vi "Read Instrument.vi"(8 "error in (no error)":errorcluster, 11 "Submodule EOL configuration in":refnum<class "Submodule EOL configuration.lvclass">) -> (0 "error out":errorcluster, 2 "Instrument":T1, 3 "Submodule EOL configuration out":refnum<class "Submodule EOL configuration.lvclass">)   [LabVIEW 2025, in "Submodule EOL.lvlib" / "Submodule EOL configuration.lvclass"]
uses:
  Submodule EOL configuration.lvclass
  Instrumnet.ctl
  Submodule EOL configuration.lvclass/Submodule EOL configuration.ctl
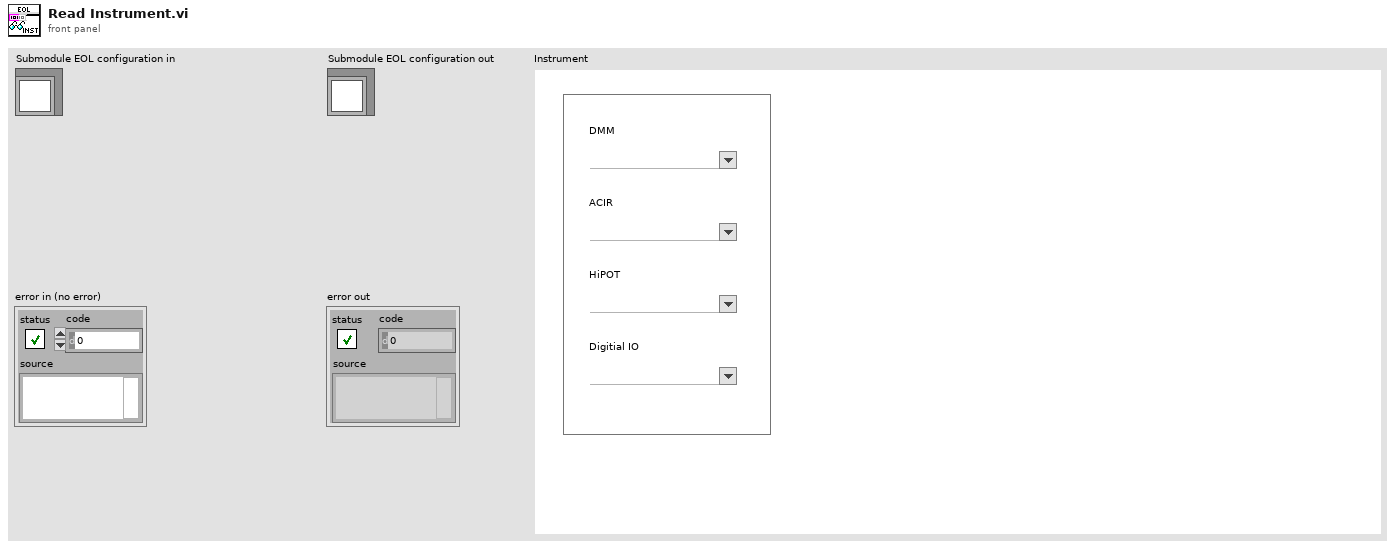
[diagram p1: front panel]
types:
  T1 = typedef "Submodule EOL.lvlib/Submodule EOL configuration.lvclass/Instrumnet.ctl" = cluster{"Digitial IO":string, "HiPOT":string, "ACIR":string, "DMM":string}
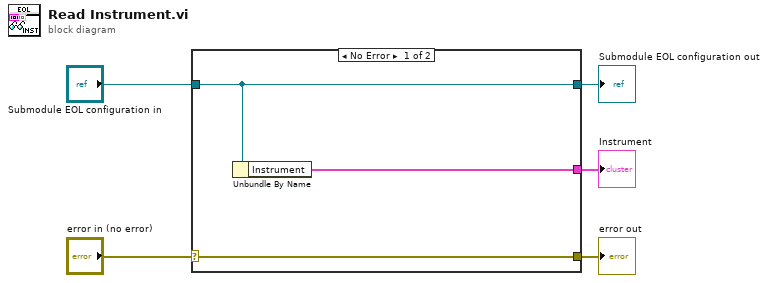
[diagram p0: block diagram]
diagram:
  n1 = case shown="No Error" "error in (no error)" {
    selector: "error in (no error)" -> [w8 w9]
    tunnel: [w8 w9] -> w4
    tunnel: [w7 w10] -> w2
    tunnel: "Submodule EOL configuration in" -> [w7 w10]
    tunnel: [w6 _] -> w1
    frame No Error {
      n2 = Unbundle By Name(w7) -> ("Instrument"=w6:T1)
    }
    frame Error {
    }
  }
  "error out" <- w4
  "Submodule EOL configuration out" <- w2
  "Instrument" <- w1
